vi "work2_cooker_draft_module.vi"() -> ()   [LabVIEW 2026]
panel:
  in  "quantity":dbl
  in  "Cook Meal":bool
  in  "Cook Burgers":bool
  in  "Stop":bool
  # "Producer Consumer Demo"
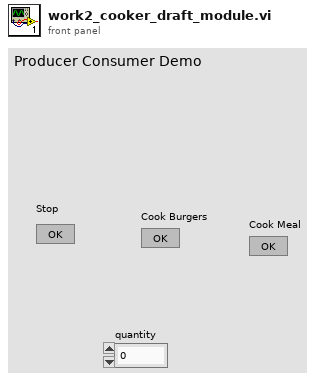
[diagram p1: front panel]
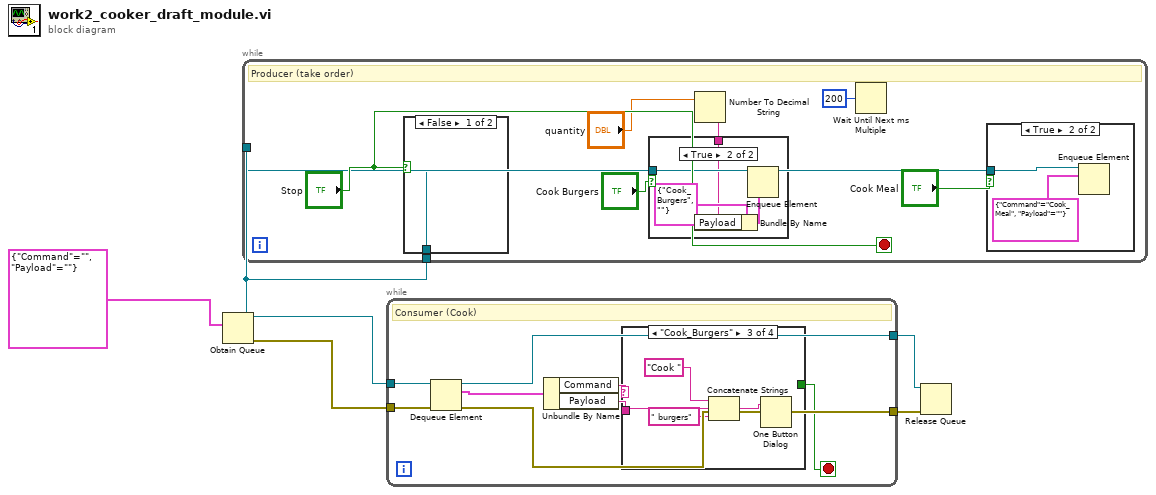
[diagram p0: block diagram]
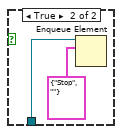
[diagram p4: hidden frame]
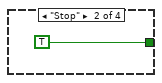
[diagram p6: hidden frame]
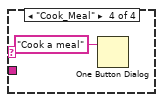
[diagram p7: hidden frame]
diagram:
  n1 = Obtain Queue(element data type=cluster{"Command":string, "Payload":string} {"Command"="", "Payload"=""}) -> (queue out=w1:refnum<queue>, error out=w5:errorcluster)  [unwired: 4 in, 1 out]
  n2 = while {
    tunnel: w1 -> [w10]
    tunnel: w1 -> [w6]
    stop <- "Stop" stop-if-true
    # "Producer (take order)"
    n3 = case shown="False" "Stop" {
      tunnel: w6 -> [_ w21]
      frame False {
      }
      frame True {
        n4 = Enqueue Element(queue=w21, element=cluster{"Command":string, "Payload":string} {"Command"="Stop", "Payload"=""}) -> ()  [unwired: 2 in, 3 out]
      }
    }
    n5 = Number To Decimal String(number="quantity") -> (decimal integer string=w9:string)  [unwired: 1 in]
    n6 = case shown="True" "Cook Burgers" {
      tunnel: w10 -> [_ w19]
      tunnel: w9 -> [_ w17]
      frame False {
      }
      frame True {
        n7 = Bundle By Name(cluster=cluster{"Command":string, "Payload":string} {"Command"="Cook_Burgers", "Payload"=""} ("element"), "Payload"=w17) -> (w16:cluster{"Command":string, "Payload":string})
        n8 = Enqueue Element(queue=w19, element=w16) -> ()  [unwired: 2 in, 3 out]
      }
    }
    n9 = Wait Until Next ms Multiple(millisecond multiple=u32 200) -> ()  [unwired: 1 out]
    n10 = case shown="True" "Cook Meal" {
      tunnel: w6 -> [_ w15]
      frame False {
      }
      frame True {
        n11 = Enqueue Element(queue=w15, element=cluster{"Command":string, "Payload":string} {"Command"="Cook_Meal", "Payload"=""}) -> ()  [unwired: 2 in, 3 out]
      }
    }
  }
  n12 = while {
    tunnel: w1 -> [w29]
    tunnel: w5 -> [w28]
    tunnel: [w27] -> w4
    tunnel: [w26] -> w3
    stop <- w22 stop-if-true
    # "Consumer (Cook)"
    n13 = Dequeue Element(queue=w29, error in (no error)=w28) -> (queue out=w27:refnum<queue>, element=w25:cluster{"Command":string, "Payload":string}, error out=w26:errorcluster)  [unwired: 1 in, 1 out]
    n14 = Unbundle By Name(w25) -> ("Command"=w24:string, "Payload"=w23:string)
    n15 = case shown="\"Cook_Burgers\"" w24 {
      tunnel: w23 -> [_ _ w33 _]
      tunnel: [_ TRUE _ _] -> w22
      frame Default {
      }
      frame "Stop" {
      }
      frame "Cook_Burgers" {
        n16 = Concatenate Strings("Cook " ("string"), w33, " burgers" ("string")) -> (w31:string)
        n17 = One Button Dialog(message=w31) -> ()  [unwired: 1 in, 1 out]
      }
      frame "Cook_Meal" {
        n18 = One Button Dialog(message="Cook a meal") -> ()  [unwired: 1 in, 1 out]
      }
    }
  }
  n19 = Release Queue(queue=w4, error in (no error)=w3) -> ()  [unwired: 1 in, 3 out]
